vi "IDS Preview Capture.vi"(4 "No Bin Image Ref":T1, 6 "Pixel Size (µm)":dbl=-1.0, 8 "Image Ref":T1, 9 "IDS Camera Ref":refnum<k24>, 10 "IDS Actions":T2, 11 "IDS Notifier":refnum<notifier>) -> (0 "Error":errorcluster, 3 "IDS Notifier":refnum<notifier>)   [LabVIEW 2021]
uses:
  IDS Controls/IDS Actions.ctl
  IDS Controls/IDS Notifier Element.ctl
  IDS Controls/IDS Parameters.ctl
  IDS Controls/IDS Parameter List.ctl
  IDS Controls/IDS ROI.ctl
  <vilib>/vision/Image Controls.llb/IMAQ Image.ctl
  C:/Users/Ries Lab/Documents/Microscope Control from Sheng Account/Microscope-Control/Device Library/Cameras/IDS/IDS LabView Examples/LabVIEW/ueye.NET/uEyeDotNet.dll
  IDS LabView Examples/LabVIEW/ueye.NET/uEyeDotNet.dll
  Tools/TIFF Image Read and Write/ImageJ TIF Type Defs/TIF Write Image Information.ctl
  Camera Controls/Camera IMAQ Key Info.ctl
  <vilib>/vision/NI_Vision_Development_Module.lvlib
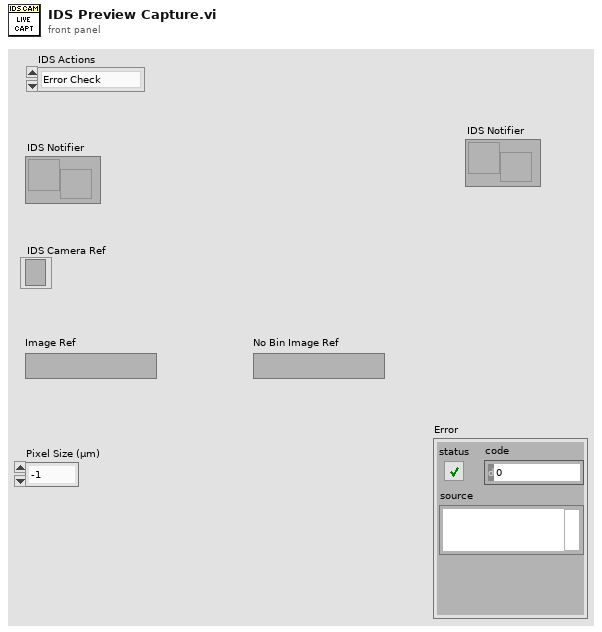
[diagram p1: front panel]
types:
  T1 = typedef "IMAQ Image.ctl" = refnum<image>
  T2 = typedef "IDS Actions.ctl" = enum16{"Error Check", "Initialize", "Preview", "Record", "Abort", "Record Settings", "Set Parameter", "Get Parameter", "Set ROI", "Get ROI", "Status", "Quit"}
  T3 = typedef "Camera IMAQ Key Info.ctl" = cluster{"Frame":u32, "Sensor Height":i32, "Sensor Width":i32, "ROI Height":i32, "ROI Width":i32, "ROI Enable?":bool, "Bit per Pixel":u8}
  T4 = typedef "TIF Write Image Information.ctl" = cluster{"Image Width (Pixels)":u32, "Image Height (Pixels)":u32, "Pixel Width (µm)":dbl, "Pixel Height (µm)":dbl, "Bits Per Sample (e.g. 16)":u32, "No. of Frames":u32, "No. of Slices":u32, "Time Step (sec)":dbl, "Z Step (µm)":dbl}
  T5 = typedef "IDS Notifier Element.ctl" = cluster{"IDS Actions":T2, "Received?":bool, "IDS Parameter":T6, "IDS ROI":T8, "Running?":bool, "File Path":path, "# of frames":u32, "Image Ref":T1, "Error":errorcluster, "Binning":i32}
  T6 = typedef "IDS Parameters.ctl" = cluster{"Parameter":T7, "Value":dbl}
  T7 = typedef "IDS Parameter List.ctl" = enum16{"Exposure Time (s)", "Binning"}
  T8 = typedef "IDS ROI.ctl" = cluster{"H Offset":i32, "V Offset":i32, "H Width":i32, "V Width":i32}
  T9 = enum16{"big-endian, network order", "native, host order", "little-endian"}
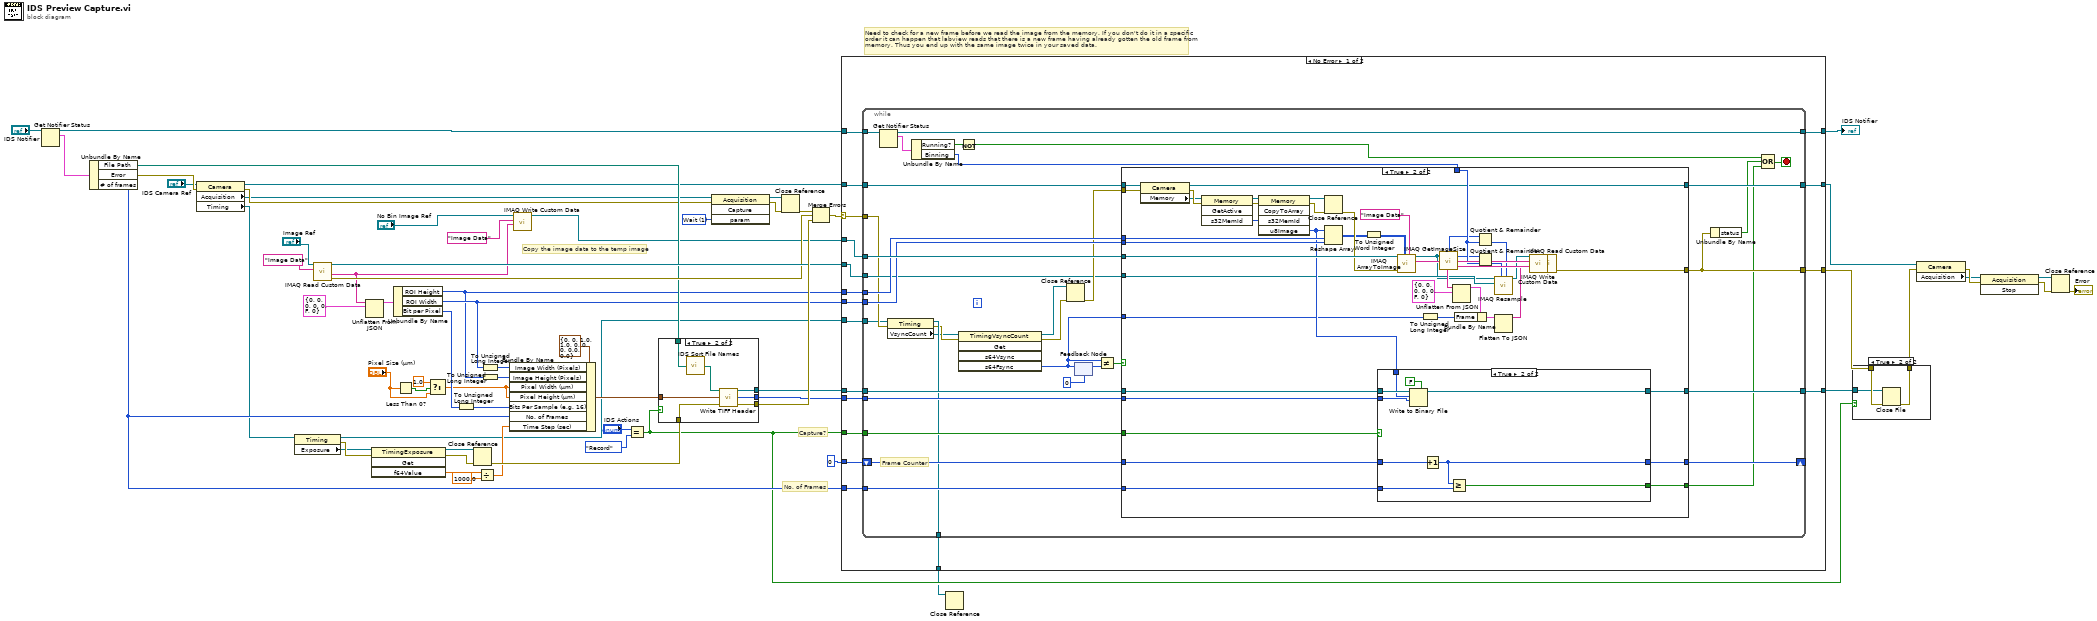
[diagram p0: block diagram]
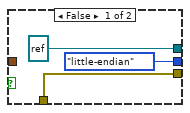
[diagram p3: hidden frame]
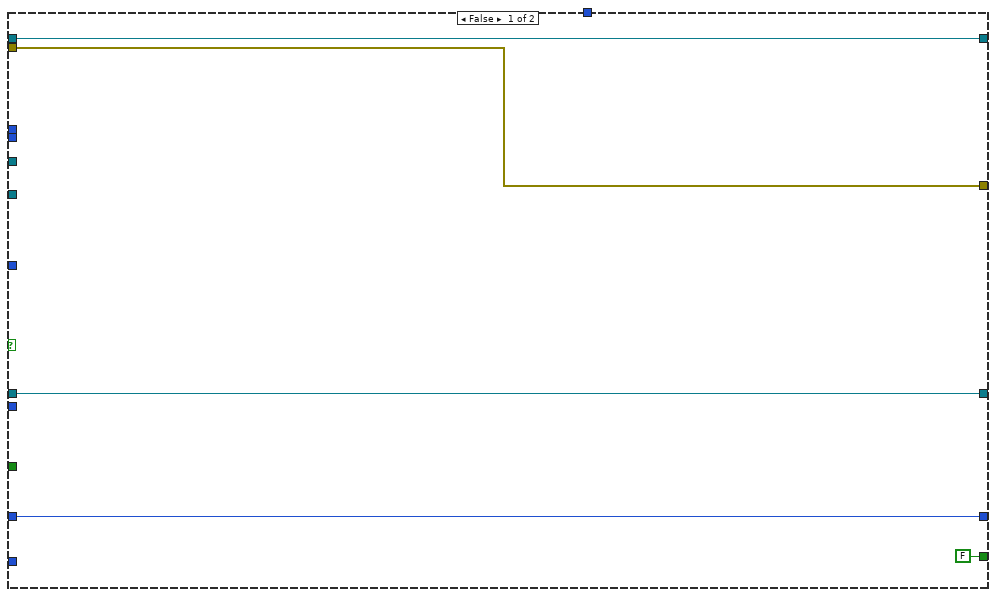
[diagram p4: hidden frame]
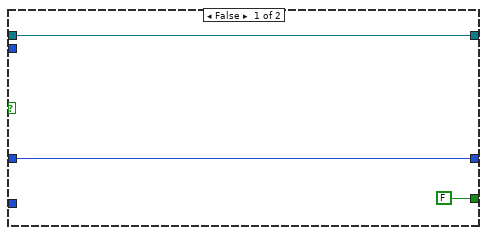
[diagram p5: hidden frame]
diagram:
  w27 = 1 items=["DontWait"=0, "Wait"=1, "Force"=16384] ("param")
  # "Copy the image data to the temp image"
  # "Need to check for a new frame before we read the image from the memory. If you don't do it in a specific\norder it can happen that labview reads that there is a new frame having already gotten the old frame from\nmemory. Thus you end up with the same image twice in your saved data."
  # "Capture?"
  # "No. of Frames"
  n1 = Get Notifier Status(notifier="IDS Notifier") -> (notifier out=w54:refnum<notifier>, current notification=w53:T5)  [unwired: 1 in, 3 out]
  n2 = Unbundle By Name(w53) -> ("File Path"=w34:path, "Error"=w7:errorcluster, "# of frames"=w35:u32)
  n3 = property class="Camera"(reference="IDS Camera Ref", error in=w7) -> (reference out=w11:refnum<k24>, error out=w10:errorcluster, "Acquisition"=w9:refnum<k24>, "Timing"=w8:refnum<k24>)
  n4 = property class="Timing"(reference=w8) -> (reference out=w14:refnum<k24>, error out=w13:errorcluster, "Exposure"=w12:refnum<k24>)  [unwired: 1 in]
  n5 = call "IMAQ Read Custom Data"("Key"="Image Data", "Image"="Image Ref") -> ("error out"=w41:errorcluster, "Custom Data Out"=w39:string, "Image (duplicate)"=w42:T1)  [unwired: 7 in]
  n6 = Unflatten From JSON(JSON string=w39, type and defaults=T3 {"Frame"=0, "Sensor Height"=0, "Sensor Width"=0, "ROI Height"=0, "ROI Width"=0, "ROI Enable?"=FALSE, "Bit per Pixel"=0} ("Camera IMAQ Key Info")) -> (value=w38:T3)  [unwired: 5 in, 1 out]
  n7 = invoke class="TimingExposure" method="Get"(reference=w12, error in=w13) -> (reference out=w45:refnum<k24>, error out=w44:errorcluster, "f64Value"=w24:dbl)  [unwired: 2 in, 1 out]
  n8 = Unbundle By Name(w38) -> ("ROI Height"=w32:i32, "ROI Width"=w33:i32, "Bit per Pixel"=w26:u8)
  n9 = Less Than 0?(x="Pixel Size (µm)") -> (x < 0?=w19:bool)
  n10 = Select(t=1.0, s=w19, f="Pixel Size (µm)") -> (s? t:f=w20:dbl)
  n11 = To Unsigned Long Integer(number=w26) -> (unsigned 32bit integer=w21:u32)
  n12 = Close Reference(reference=w45, error in (no error)=w44) -> (error out=w43:errorcluster)
  n13 = Divide(x=w24, y=1000.0) -> (x/y=w22:dbl)
  n14 = To Unsigned Long Integer(number=w33) -> (unsigned 32bit integer=w48:u32)
  n15 = To Unsigned Long Integer(number=w32) -> (unsigned 32bit integer=w47:u32)
  n16 = Bundle By Name(cluster=T4 {"Image Width (Pixels)"=0, "Image Height (Pixels)"=0, "Pixel Width (µm)"=1.0, "Pixel Height (µm)"=1.0, "Bits Per Sample (e.g. 16)"=0, "No. of Frames"=0, "No. of Slices"=0, "Time Step (sec)"=0.0, "Z Step (µm)"=0.0} ("Image Info"), "Image Width (Pixels)"=w48, "Image Height (Pixels)"=w47, "Pixel Width (µm)"=w20, "Pixel Height (µm)"=w20, "Bits Per Sample (e.g. 16)"=w21, "No. of Frames"=w35, "Time Step (sec)"=w22) -> (w49:T4)
  n17 = call "IMAQ Write Custom Data"("Custom Data In"=w39, "Key"="Image Data", "Image"="No Bin Image Ref") -> ("Image Out"=w16:T1)  [unwired: 7 in, 1 out]
  n18 = Equal?(x="IDS Actions", y=IDS_Actions."Record") -> (x = y?=w29:bool)
  n19 = case shown="True" w29 {
    tunnel: w49 -> [_ w75]
    tunnel: w34 -> [_ w70]
    tunnel: [w68 w74] -> w46
    tunnel: w43 -> [w68 w73]
    tunnel: [refnum<file> refnum ("File Ref") w72] -> w36
    tunnel: [T9."little-endian" ("Byte Order") w71] -> w37
    frame False {
    }
    frame True {
      n20 = call "IDS Sort File Names.vi"("Requested File Path"=w70) -> ("Resulting File Path"=w69:path)  [unwired: 14 in]
      n21 = call "Write TIFF Header.vi"("File Path"=w69, "Image Info"=w75, "Error"=w73) -> ("File Ref"=w72:refnum<file>, "Byte Order"=w71:T9, "Error"=w74:errorcluster)  [unwired: 10 in]
    }
  }
  n22 = invoke class="Acquisition" method="Capture"(reference=w9, error in=w10, "param"=w27) -> (reference out=w65:refnum<k24>, error out=w64:errorcluster)  [unwired: 1 in, 2 out]
  n23 = Close Reference(reference=w65, error in (no error)=w64) -> (error out=w63:errorcluster)
  n24 = Merge Errors(w63, w41, w46) -> (w62:errorcluster)
  n25 = case shown="No Error" w62 {
    selector: w62 -> [w89 w194]
    tunnel: w54 -> [w93 w192]
    tunnel: [w88 w192] -> w57
    tunnel: w11 -> [w92 w193]
    tunnel: w32 -> [w91 _]
    tunnel: w33 -> [w90 _]
    tunnel: w42 -> [w77 _]
    tunnel: [w87 w194] -> w30
    tunnel: [w86 w193] -> w2
    tunnel: w29 -> [w85 _]
    tunnel: w37 -> [w84 _]
    tunnel: w36 -> [w83 w191]
    tunnel: w35 -> [w82 _]
    tunnel: [w81 w191] -> w31
    tunnel: w14 -> [w80 w190]
    tunnel: [w79 w190] -> w28
    tunnel: u32 0 ("s64Fsync") -> [w78 _]
    tunnel: w16 -> [w76 _]
    frame No Error {
      n26 = while {
        tunnel: w93 -> [w128]
        tunnel: w92 -> [w127]
        tunnel: w91 -> [w124]
        tunnel: w90 -> [w123]
        tunnel: w89 -> [w95]
        tunnel: [w126] -> w86
        tunnel: w76 -> [w125]
        tunnel: [w122] -> w88
        tunnel: [w121] -> w87
        tunnel: w85 -> [w107]
        tunnel: w84 -> [w118]
        tunnel: w83 -> [w119]
        tunnel: w82 -> [w120]
        tunnel: [w114] -> w81
        tunnel: w80 -> [w94]
        tunnel: [w98] -> w79
        shift-right: [w109] -> _
        shift-left: w78 -> [w110]
        tunnel: w77 -> [w102]
        stop <- w115 stop-if-true
        # "Frame Counter"
        n27 = Get Notifier Status(notifier=w128) -> (notifier out=w122:refnum<notifier>, current notification=w99:T5)  [unwired: 1 in, 3 out]
        n28 = property class="Timing"(reference=w94, error in=w95) -> (reference out=w98:refnum<k24>, error out=w97:errorcluster, "VsyncCount"=w96:refnum<k24>)
        n29 = Unbundle By Name(w99) -> ("Running?"=w101:bool, "Binning"=w100:i32)
        n30 = invoke class="TimingVsyncCount" method="Get"(reference=w96, error in=w97) -> (reference out=w103:refnum<k24>, error out=w105:errorcluster, "s64Fsync"=w111:i64)  [unwired: 3 in, 2 out]
        n31 = Not(x=w101) -> (.not. x?=w117:bool)
        n32 = Close Reference(reference=w103, error in (no error)=w105) -> (error out=w104:errorcluster)
        n33 = feedback #1(i64 0 ("s64Fsync")) -> (w112:i64)
        n34 = feedback-in #1(w111) -> ()
        n35 = Not Equal?(x=w111, y=w112) -> (x != y?=w106:bool)
        n36 = case shown="True" w106 {
          tunnel: w127 -> [w133 w134]
          tunnel: [w133 w138] -> w126
          tunnel: w125 -> [_ w172]
          tunnel: w124 -> [_ w171]
          tunnel: w123 -> [_ w170]
          tunnel: [w132 w168] -> w121
          tunnel: w120 -> [_ w159]
          tunnel: w119 -> [w129 w158]
          tunnel: w118 -> [_ w157]
          tunnel: [w129 w153] -> w114
          tunnel: w111 -> [_ w151]
          tunnel: w104 -> [w132 w135]
          tunnel: w110 -> [w131 w150]
          tunnel: [w131 w149] -> w109
          tunnel: [FALSE w148] -> w108
          tunnel: w107 -> [_ w147]
          tunnel: w102 -> [_ w146]
          tunnel: w100 -> [_ w143]
          frame False {
          }
          frame True {
            w165 = "Image Data" ("Key")
            n37 = property class="Camera"(reference=w134, error in=w135) -> (reference out=w138:refnum<k24>, error out=w137:errorcluster, "Memory"=w136:refnum<k24>)
            n38 = invoke class="Memory" method="GetActive"(reference=w136, error in=w137) -> (reference out=w177:refnum<k24>, error out=w175:errorcluster, "s32MemId"=w176:i32)  [unwired: 2 in, 1 out]
            n39 = invoke class="Memory" method="CopyToArray"(reference=w177, error in=w175, "s32MemId"=w176) -> (reference out=w174:refnum<k24>, error out=w173:errorcluster, "u8Image"=w154:u8[])  [unwired: 2 in, 2 out]
            n40 = Close Reference(reference=w174, error in (no error)=w173) -> (error out=w169:errorcluster)
            n41 = Reshape Array(w154, w171, w170) -> (w155:u8[][])
            n42 = To Unsigned Word Integer(number=w155) -> (unsigned 16bit integer=w156:u16[][])
            n43 = case shown="True" w147 {
              tunnel: w159 -> [_ w189]
              tunnel: w158 -> [w180 w185]
              tunnel: w157 -> [_ w188]
              tunnel: [w180 w186] -> w153
              tunnel: w154 -> [_ w184]
              tunnel: w150 -> [w179 w183]
              tunnel: [w179 w182] -> w149
              tunnel: [FALSE w181] -> w148
              frame False {
              }
              frame True {
                n44 = Write to Binary File(file (use dialog)=w185, data=w184, 5:FALSE ("prepend array or string size? (T)"), 9:w188) -> (refnum out=w186:refnum<file>)  [unwired: 2 in, 2 out]
                n45 = Increment(x=w183) -> (x+1=w182:u32)
                n46 = Greater Or Equal?(x=w182, y=w189) -> (x >= y?=w181:bool)
              }
            }
            n47 = call "IMAQ ArrayToImage"("Image Pixels (U16)"=w156, "error in (no error)"=w169, "Image"=w172) -> ("Image Out"=w139:T1)  [unwired: 7 in, 1 out]
            n48 = To Unsigned Long Integer(number=w151) -> (unsigned 32bit integer=w152:u32)
            n49 = call "IMAQ GetImageSize"("Image"=w139) -> ("Y Resolution"=w141:i32, "X Resolution"=w140:i32)  [unwired: 3 in, 1 out]
            n50 = Quotient & Remainder(x=w140, y=w143) -> (floor(x/y)=w144:i32)  [unwired: 1 out]
            n51 = Quotient & Remainder(x=w141, y=w143) -> (floor(x/y)=w142:i32)  [unwired: 1 out]
            n52 = call "IMAQ Resample"("X Resolution"=w144, "Y Resolution"=w142, "Image Dst"=w146, "Image Src"=w139) -> ("Image Dst Out"=w145:T1)  [unwired: 6 in, 1 out]
            n53 = call "IMAQ Read Custom Data"("Key"=w165, "Image"=w145) -> ("error out"=w166:errorcluster, "Custom Data Out"=w164:string, "Image (duplicate)"=w167:T1)  [unwired: 7 in]
            n54 = Unflatten From JSON(JSON string=w164, type and defaults=T3 {"Frame"=0, "Sensor Height"=0, "Sensor Width"=0, "ROI Height"=0, "ROI Width"=0, "ROI Enable?"=FALSE, "Bit per Pixel"=0} ("Camera IMAQ Key Info")) -> (value=w162:T3)  [unwired: 5 in, 1 out]
            n55 = Bundle By Name(cluster=w162, "Frame"=w152) -> (w161:T3)
            n56 = Flatten To JSON(anything=w161) -> (JSON string=w160:string)  [unwired: 2 in, 1 out]
            n57 = call "IMAQ Write Custom Data"("error in (no error)"=w166, "Custom Data In"=w160, "Key"=w165, "Image"=w167) -> ("error out"=w168:errorcluster)  [unwired: 6 in, 1 out]
          }
        }
        n58 = Unbundle By Name(w121) -> ("status"=w116:bool)
        n59 = Compound Arithmetic op=OR(w117, w116, w108) -> (w115:bool)
      }
    }
    frame Error {
    }
  }
  "IDS Notifier" <- w57
  n60 = Close Reference(reference=w28) -> ()  [unwired: 1 in, 1 out]
  n61 = case shown="True" w29 {
    tunnel: w31 -> [_ w196]
    tunnel: w30 -> [w195 w198]
    tunnel: [w195 w197] -> w3
    frame False {
    }
    frame True {
      n62 = Close File(refnum=w196, error in=w198) -> (error out=w197:errorcluster)  [unwired: 1 out]
    }
  }
  n63 = property class="Camera"(reference=w2, error in=w3) -> (error out=w5:errorcluster, "Acquisition"=w4:refnum<k24>)  [unwired: 1 out]
  n64 = invoke class="Acquisition" method="Stop"(reference=w4, error in=w5) -> (reference out=w60:refnum<k24>, error out=w59:errorcluster)  [unwired: 1 in, 1 out]
  n65 = Close Reference(reference=w60, error in (no error)=w59) -> (error out=→"Error":errorcluster)
